vi "TEST - Merge Directories.vi"(8 "error in (no error)":errorcluster) -> (0 "error out":errorcluster, 2 "pass":bool)   [LabVIEW 2020]
uses:
  <userlib>/_OpenG.lib/error/error.llb/openg_error.lvlib
  source/library/openg_file.lvlib
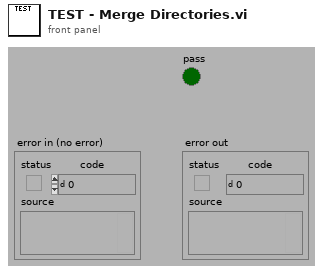
[diagram p1: front panel]
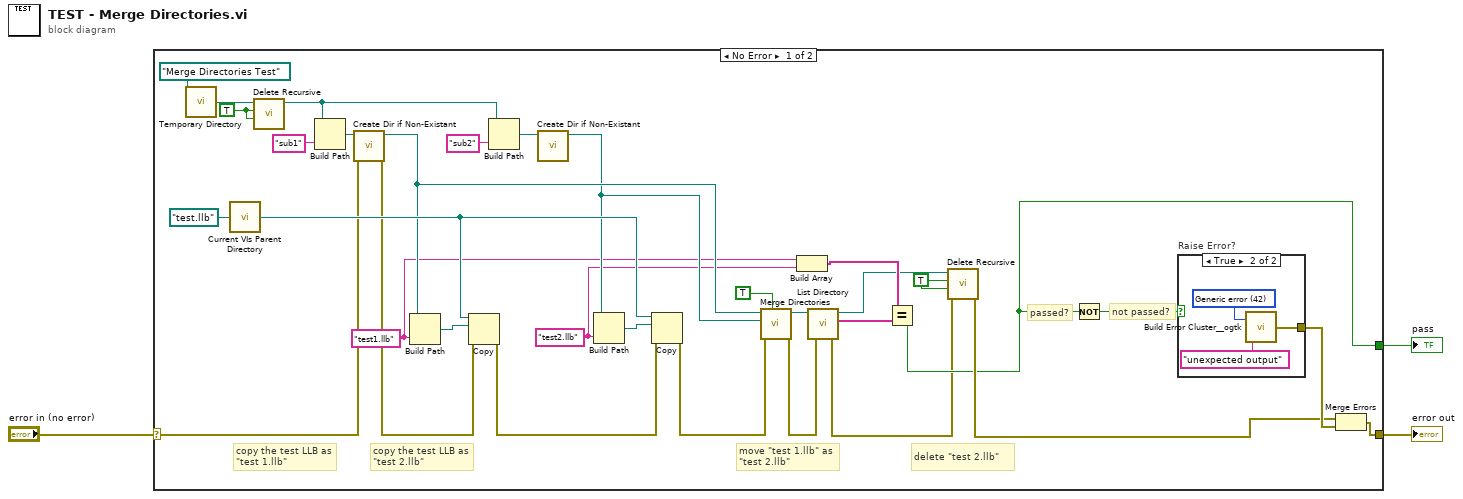
[diagram p0: block diagram]
diagram:
  n1 = case shown="No Error" "error in (no error)" {
    selector: "error in (no error)" -> [w20 w40]
    tunnel: [w29 _] -> w3
    tunnel: [w36 w40] -> w1
    frame No Error {
      w4 = TRUE ("Recursive? (FALSE)")
      w6 = TRUE ("Recursive? (FALSE)")
      w12 = "test1.llb" ("name or relative path")
      w11 = "test2.llb" ("name or relative path")
      # "delete \"test 2.llb\""
      # "move \"test 1.llb\" as \"test 2.llb\""
      # "copy the test LLB as \"test 2.llb\""
      # "copy the test LLB as \"test 1.llb\""
      # "not passed?"
      # "passed?"
      n2 = call "Temporary Directory.vi"("Relative path (.)"=path "Merge Directories Test") -> ("Temporary Directory (+ Relative)"=w27:path)
      n3 = call "Current VIs Parent Directory.vi"("Relative path (.)"=path "test.llb") -> ("Parent Directory (+ Relative)"=w30:path)  [unwired: 4 in]
      n4 = call "Delete Recursive.vi"("Ignore Read-Only? (FALSE)"=w4, "Recursive? (FALSE)"=w4, "Path"=w27) -> ("dup Path"=w24:path)  [unwired: 7 in, 1 out]
      n5 = Build Path(base path=w24, name or relative path="sub1") -> (appended path=w23:path)
      n6 = call "Create Dir if Non-Existant.vi"("error in (no error)"=w20, "Directory Path"=w23) -> ("error out"=w21:errorcluster, "dup Directory Path"=w17:path)  [unwired: 7 in, 1 out]
      n7 = Build Path(base path=w17, name or relative path=w12) -> (appended path=w19:path)
      n8 = Copy(8:w21, 10:w19, 11:w30) -> (0:w31:errorcluster)  [unwired: 2 in, 2 out]
      n9 = Build Path(base path=w24, name or relative path="sub2") -> (appended path=w22:path)
      n10 = call "Create Dir if Non-Existant.vi"("Directory Path"=w22) -> ("dup Directory Path"=w16:path)  [unwired: 8 in, 2 out]
      n11 = Build Path(base path=w16, name or relative path=w11) -> (appended path=w18:path)
      n12 = Copy(8:w31, 10:w18, 11:w30) -> (0:w15:errorcluster)  [unwired: 2 in, 2 out]
      n13 = call "Merge Directories.vi"("Delete Source? (FALSE)"=TRUE, "error in (no error)"=w15, "target directory path"=w16, "source directory path"=w17) -> ("error out"=w10:errorcluster, "dup target directory path"=w13:path)  [unwired: 6 in]
      n14 = Build Array(w12, w11) -> (w8:string[])
      n15 = call "List Directory.vi"("error in (no error)"=w10, "directory path"=w13) -> ("error out"=w5:errorcluster, "file names"=w9:string[], "dup directory path"=w7:path)  [unwired: 2 in, 1 out]
      n16 = Equal?(x=w8, y=w9) -> (x = y?=w29:bool)
      n17 = call "Delete Recursive.vi"("error in (no error)"=w5, "Ignore Read-Only? (FALSE)"=w6, "Recursive? (FALSE)"=w6, "Path"=w7) -> ("error out"=w33:errorcluster)  [unwired: 6 in, 1 out]
      n18 = Not(x=w29) -> (.not. x?=w34:bool)
      n19 = case "Raise Error?" shown="True" w34 {
        tunnel: [_ w37] -> w35
        frame False {
        }
        frame True {
          w38 = 42 items=["No error", "Argument error", "Memory is full", "Out of zone", "End of file", "File already open", "Generic file I/O error", "File not found", "File permission error", "Disk is full", "Duplicate path", "Too many files open", "System feature not enabled", "Resource file not found", "Cannot add resource", "Resource not found", "Image not found", "Image memory error", "Pen does not exist", "Config type invalid", "Config token not found", "Config parse error", "Config memory error", "Bad external code format", "Bad external code offset", "External code not present", "Null window", "Destroy window error", "Null menu", "Print aborted", "Bad print record", "Print driver error", "Windows error during printing", "Memory error during printing", "Print dialog error", "Generic print error", "Invalid device refnum", "Device not found", "Device parameter error", "Device unit error", "Cannot open device", "Device call aborted", "Generic error", "Cancelled by user", "Object ID too low", "Object ID too high", "Object not in heap", "Unknown heap", "Unknown object (invalid DefProc)", "Unknown object (DefProc not in table)", "Message out of range", "Invalid (null) method", "Unknown message", "Manager call not supported", "Bad address", "Network operation in progress", "Network operation timed out", "Connection is busy", "Network attribute not supported", "Network error", "Address in use", "System out of memory", "Connection aborted", "Connection refused", "Not connected", "Already connected", "Connection closed", "Initialization error (interapplication manager)", "Bad occurrence", "Wait on unbound occurrence handler", "Occurrence queue overflow", "Datalog type conflict", "Unused", "Unrecognized type (interapplication manager)", "Memory corrupt", "Failed to make temporary DLL", "Old CIN version", "Drag socket not found", "Failed to load drop-object", "Failed to register OLE object", "Failed to release OLE object", "Format specifier type mismatch", "Unknown format specifier", "Too few format specifiers", "Too many format specifiers", "Scan failed", "Newer CIN version", "Error converting to variant", "Runtime menu error", "Password tampered", "Variant attribute not found", "Incompatible variant data type", "Event data is not available", "Event Store is not present", "Occurrence is not found", "Event Queue is not created", "Event info is not available", "Refnum passed is NULL", "Error retrieving Class GUID", "Error retrieving CoClass GUID", "Error retrieving TypeLib GUID.", "Bad built application magic bytes.", "Specific driver is different from the specific driver associated with the Logical Name.", "There is no session opened to the class driver.", "Max Error", "MAX - Error with config objects", "MAX - Error loading configuration", "MAX - Group not supported"]
          n20 = call <userlib>:"Build Error Cluster__ogtk.vi"("String to Prepend to source (\"\")"="unexpected output" ("String to Prepend to source (\"\")"), "code"=w38) -> ("error out"=w37:errorcluster)
        }
      }
      n21 = Merge Errors(w33, w35) -> (w36:errorcluster)
    }
    frame Error {
    }
  }
  "pass" <- w3
  "error out" <- w1
